vi "generate default line.vi"(8 "error in":errorcluster, 10 "Last Line In":T1, 11 "objects in":T2) -> (0 "error out":errorcluster, 2 "Line out":T1, 3 "objects out":T2)   [LabVIEW 2015, in "Scan Engine editor node.lvclass"]
uses:
  Scan Engine editor node.lvclass
  configuration/Line.ctl
  <vilib>/NI/Tag Bus Module Framework/channel/TBM channel.lvclass
  <vilib>/NI/DCAF/Tag Editor Core/Table API/Table Manager/object ref.ctl
  <vilib>/NI/DCAF/Tag Editor Core/Configuration Editor/Classes/Engine Parent/Engine Parent Editor Node.lvclass
  <vilib>/NI/DCAF/Tag Editor Core/Configuration Editor/Classes/Module editor node/module editor node.lvclass
  configuration/Scan Engine configuration.lvclass
  <vilib>/NI/Tag Bus/tag/tag descriptor.lvclass/tag descriptor.ctl
  <vilib>/NI/Tag Bus Module Framework/channel/TBM channel.lvclass/TBM channel.ctl
  <vilib>/NI/Tag Bus/tag/Data Type.ctl
  configuration/permissions.ctl
  <vilib>/NI/Tag Bus/tag/read data type.vi
  <vilib>/NI/Tag Bus Module Framework/channel/Read channel classification.vi
  <vilib>/NI/Configuration Framework/serializable configuration/NISE_CEF_serializable configuration.lvclass
  <vilib>/NI/Tag Bus/tag/tag descriptor.lvclass
  <vilib>/NI/DCAF/Tag Editor Core/Table API/Table Manager/Table Manager.lvclass
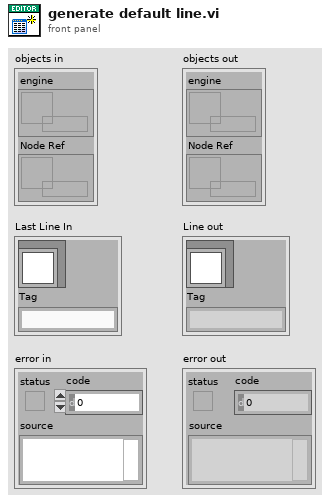
[diagram p1: front panel]
types:
  T1 = typedef "Scan Engine configuration.lvclass/Line.ctl" = cluster{"channel":refnum<class "TBM channel.lvclass">, "Tag":string}
  T2 = typedef "Table Manager.lvlib/Table Manager.lvclass/object ref.ctl" = cluster{"engine":refnum<data-value>, "Node Ref":refnum<data-value>}
  T3 = typedef "tag bus.lvlib/tag descriptor.lvclass/Data Type.ctl" = enum16{"Double", "Single", "I64", "I32", "I16", "I8", "U64", "U32", "U16", "U8", "Boolean", "String", "Array of Double", "Array of Single", "Array of I64", "Array of I32", "Array of I16", "Array of I8", "Array of U64", "Array of U32", "Array of U16", "Array of U8", "Array of Boolean", "Array of String"}
  T4 = typedef "TBM channel.lvclass/channel classification.ctl" = enum16{"input data", "output data", "processing parameter", "processing result"}
  T5 = typedef "Scan Engine configuration.lvclass/permissions.ctl" = enum32{"Read from HW", "Write to HW"}
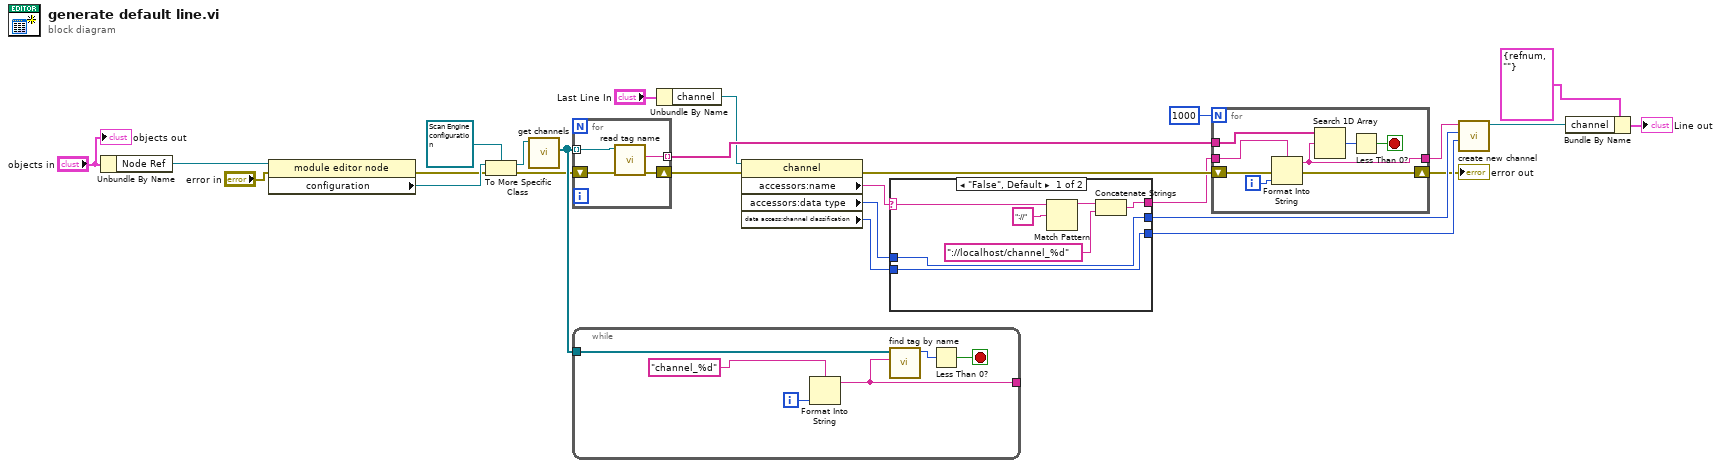
[diagram p0: block diagram]
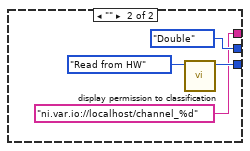
[diagram p2: hidden frame]
diagram:
  n1 = Unbundle By Name("objects in") -> ("Node Ref"=w24:refnum<data-value>)
  n2 = property class="module editor node"(reference=w24, error in="error in") -> (error out=w19:errorcluster, "configuration"=w23:refnum<class "NISE_CEF_serializable configuration.lvclass">)  [unwired: 1 out]
  n3 = To More Specific Class(target class=refnum<class "Scan Engine configuration.lvclass"> refnum ("module configuration in"), reference=w23, error in=w19) -> (specific class reference=w22:refnum<class "Scan Engine configuration.lvclass">, error out=w4:errorcluster)
  n4 = call-dynamic "get channels.vi"("Scan Engine configuration in"=w22) -> ("channels"=w14:refnum<class "TBM channel.lvclass">[])  [unwired: 9 in, 1 out]
  n5 = for {
    tunnel: [w30] -> w15 mode=indexing
    tunnel: w14 -> [w29] mode=indexing
    shift-right: [w27] -> w3
    shift-left: w4 -> [w28]
    n6 = call <vilib>:"read tag name.vi"("error in"=w28, "system tag in"=w29) -> ("error out"=w27:errorcluster, "name"=w30:string)  [unwired: 7 in, 1 out]
  }
  n7 = while {
    tunnel: [w33] -> _
    tunnel: w14 -> [w34]
    i -> [w36]
    stop <- w31 stop-if-true
    n8 = Format Into String(format string="channel_%d", w36) -> (resulting string=w33:string)  [unwired: 2 in, 1 out]
    n9 = call <vilib>:"find tag by name.vi"("name"=w33, "tags in"=w34) -> ("index"=w32:i32)  [unwired: 9 in]
    n10 = Less Than 0?(x=w32) -> (x < 0?=w31:bool)
  }
  n11 = Unbundle By Name("Last Line In") -> ("channel"=w8:refnum<class "TBM channel.lvclass">)
  n12 = property class="channel"(reference=w8, error in=w3) -> (error out=w2:errorcluster, "accessors:name"=w13:string, "accessors:data type"=w11:T3, "data access:channel classification"=w10:T4)  [unwired: 1 out]
  n13 = case shown="\"False\", Default" w13 {
    selector: w13 -> [w40 _]
    tunnel: [w42 w45] -> w6
    tunnel: [w43 Data_Type."Double" ("data type")] -> w7
    tunnel: w11 -> [w43 _]
    tunnel: w10 -> [w42 _]
    tunnel: [w37 "ni.var.io://localhost/channel_%d" ("format string")] -> w1
    frame "False", Default {
      n14 = Match Pattern(string=w40, regular expression="://") -> (before substring=w39:string)  [unwired: 1 in, 3 out]
      n15 = Concatenate Strings(w39, "://localhost/channel_%d" ("format string")) -> (w37:string)
    }
    frame "" {
      n16 = call "display permission to classification.vi"("display permissions"=permissions."Read from HW") -> ("channel classification"=w45:T4)  [unwired: 10 in]
    }
  }
  n17 = for {
    N: 1000 -> [_]
    tunnel: w15 -> [w54]
    tunnel: [w51] -> w12
    shift-right: [w49] -> w5
    shift-left: w2 -> [w50]
    tunnel: w1 -> [w48]
    i -> [w55]
    stop <- w52 stop-if-true
    n18 = Format Into String(format string=w48, error in=w50, w55) -> (resulting string=w51:string, error out=w49:errorcluster)  [unwired: 1 in]
    n19 = Search 1D Array(1D array=w54, element=w51) -> (index of element=w53:i32)  [unwired: 1 in]
    n20 = Less Than 0?(x=w53) -> (x < 0?=w52:bool)
  }
  "error out" <- w5
  n21 = call <vilib>:"create new channel.vi"("channel classification"=w6, "data type"=w7, "channel name"=w12) -> ("channel"=w25:refnum<class "TBM channel.lvclass">)  [unwired: 8 in]
  n22 = Bundle By Name(cluster=T1 {"channel"=refnum, "Tag"=""} ("Line"), "channel"=w25) -> (→"Line out":T1)
  "objects out" <- "objects in"
